vi "VM3 - Read Variables (STR).vi"(6 "atomic (F)":bool, 7 "VC Handle":T3, 8 "error in":errorcluster, 11 "name_specs":string[](array[string])) -> (0 "error out":errorcluster, 1 "stats":T1[](array[typedef]), 2 "values out":string[](array[string]), 3 "dup name_specs":string[](array[string]), 4 "errCodes":T2[](array[typedef]) items=["No error", "Invalid variable type", "Variable not found", "Variable already exists", "Invalid context handle", "Input error", "Invalid data format", "No history attached", "History already attached", "Invalid history parameters", "Wrong variable name", "Wrong alias name", "Non-unique alias", "Alias not found", "No alias associated", "Alias already associated", "Wrong context name", "Non-unique context name", "Context name not found", "Invalid parameter", "Generic error", "Memory Full", "Unrecognized LV error", "Unknown error code"])   [LabVIEW 2021]
doc: "This VI reads multiple variables of the <b>String</b> data type. Refer to the VI Help for more details.\n\n<b>VC Handle</b> specifies the handle of the variable context. To operate on a global variable, pass -1 to this input. \n<b>name_specs</b> defines the name specifiers of the target variables; usually, a name specifier is merely a variable name (see the VI Help for more options).\n\n<b>atomic (F)</b>, if TRUE, guarantees that all variables are read in an atomic transaction. This prevents other VIs or threads from modifying the variables during execution.\n\n<b>values out</b> returns the variable values.\n\n<b>stats</b> returns additional information about the variable values, such as their Writer ID, update time, and update counter.\n\n<b>errCodes</b> returns VarMan error codes individually for each variable. If any element in this array is non-zero, the <b>error out</b> cluster returns the corresponding error description.\n\n::: CalcExpress Toolkit :::\nCopyright (c) 2000-2026 Konstantin Shifershteyn. All rights reserved."
uses:
  cetypes.llb/VarMan Variable Context Handle.ctl
  cetypes.llb/VarMan Error Code.ctl
  cetypes.llb/VarMan Variable Data Statistics.ctl
  cersrc/celveng32.dll
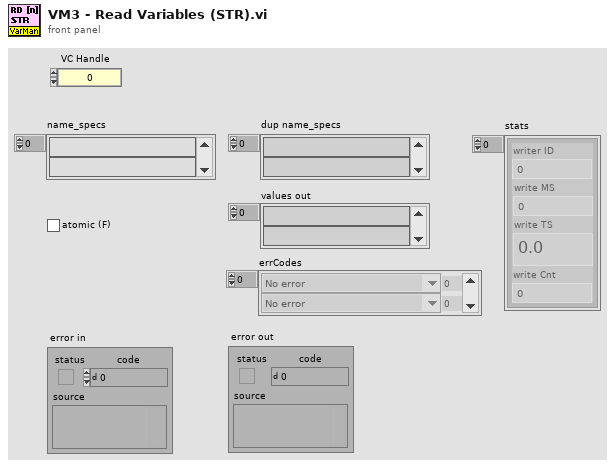
[diagram p1: front panel]
types:
  T1 = typedef "VarMan Variable Data Statistics.ctl" = cluster{"writer ID":u32, "write MS":u32, "write TS":dbl, "write Cnt":u32}
  T2 = typedef "VarMan Error Code.ctl" = u16
  T3 = typedef "VarMan Variable Context Handle.ctl" = i32
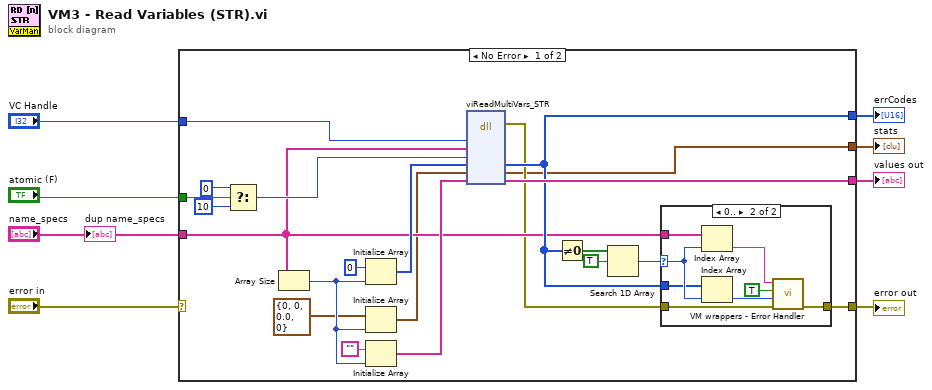
[diagram p0: block diagram]
diagram:
  n1 = case shown="No Error" "error in" {
    selector: "error in" -> [_ w39]
    tunnel: [w16 w39] -> w7
    tunnel: "VC Handle" -> [w29 _]
    tunnel: "name_specs" -> [w18 _]
    tunnel: "atomic (F)" -> [w27 _]
    tunnel: [w19 _] -> w4
    tunnel: [w20 _] -> w3
    tunnel: [w10 _] -> w1
    frame No Error {
      n2 = Select(t=0, s=w27, f=10) -> (s? t:f=w25:i32)
      n3 = Array Size(array=w18) -> (size(s)=w12:i32)
      n4 = Initialize Array(u16 0 ("element"), w12) -> (w22:u16[])
      n5 = Initialize Array(T1 {"writer ID"=0, "write MS"=0, "write TS"=0.0, "write Cnt"=0} ("stats"), w12) -> (w11:T1[])
      n6 = Initialize Array("" ("element"), w12) -> (w21:string[])
      n7 = dll-call lib="C:/LV Projects/CalcExpress 40 LV2021/vi.lib/addons/CalcExpress/cersrc/celveng*.dll" fn="viReadMultiVars_STR"("vch"=w29, "names"=w18, "lock_cycle"=w25, "errCodes"=w22, "wrStats"=w11, "strVals"=w21) -> (error out=w17:errorcluster, "errCodes"=w19:u16[], "wrStats"=w10:T1[], "strVals"=w20:string[])  [unwired: 7 in, 1 out]
      n8 = Not Equal To 0?(x=w19) -> (x != 0?=w15:bool[])
      n9 = Search 1D Array(1D array=w15, element=TRUE) -> (index of element=w13:i32)  [unwired: 1 in]
      n10 = case shown="0.." w13 {
        selector: w13 -> [_ w38]
        tunnel: w19 -> [_ w37]
        tunnel: w18 -> [_ w34]
        tunnel: w17 -> [w30 w32]
        tunnel: [w30 w31] -> w16
        frame ..-1 {
        }
        frame 0.. {
          n11 = Index Array(array=w34, index=w38) -> (element=w33:string)
          n12 = Index Array(array=w37, index=w38) -> (element=w36:u16)
          n13 = call "VM wrappers - Error Handler.vi"("error before"=w32, "VarMan error"=w36, "show name spec (F)"=TRUE, "name spec"=w33) -> ("error out"=w31:errorcluster)  [unwired: 6 in, 1 out]
        }
      }
    }
    frame Error {
    }
  }
  "error out" <- w7
  "errCodes" <- w4
  "values out" <- w3
  "stats" <- w1
  "dup name_specs" <- "name_specs"
